vi "test 1.1.0 Mutation Adds Logging Section.vi"(8 "error in (no error)":errorcluster, 11 "TestCase in":refnum<class "Mutation.lvclass">) -> (0 "error out":errorcluster, 3 "TestCase out":refnum<class "Mutation.lvclass">)   [LabVIEW 2021, in "Mutation.lvclass"]
uses:
  Mutation.lvclass
  Mutation.lvclass/Mutation.ctl
  <vilib>/addons/_JKI Toolkits/VI Tester/TestCase.llb/TestCase.lvclass
  System Explorer/Implementation/Implementation.lvlib
  Scripting/Ballard/Ballard ARINC 429 Scripting.lvlib
  C:/Program Files/National Instruments/LabVIEW 2021/vi.lib/addons/_JKI Toolkits/VI Tester/TestCase.llb/TestCase.lvclass
  C:/Dev/CustomDevice/niveristand-ballard-arinc429-custom-device/Source/Custom Device Support/Tests/Unit/Mutation/Mutation.lvclass
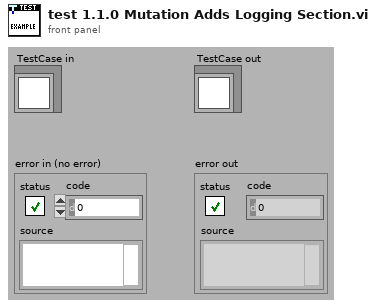
[diagram p1: front panel]
types:
  T1 = typedef "Custom Device API.lvlib/Custom Device Item Ref.ctl" = u64
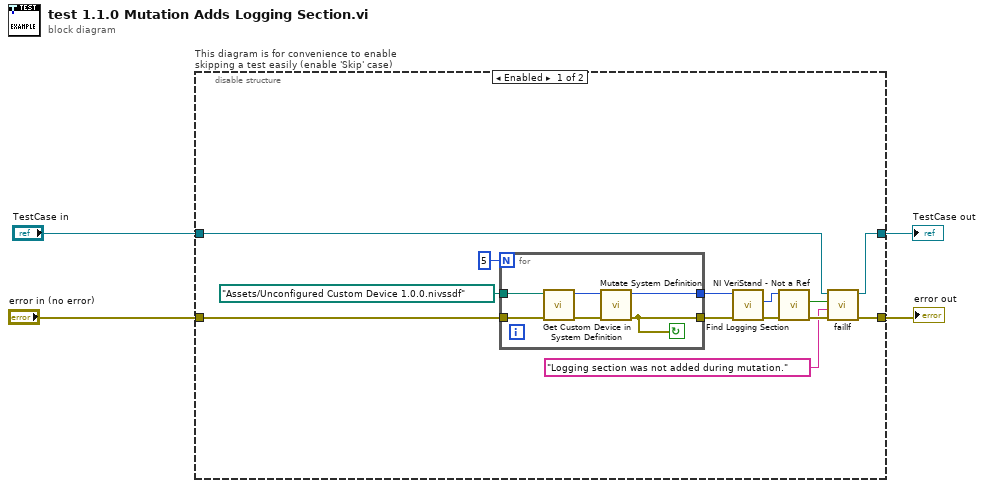
[diagram p0: block diagram]
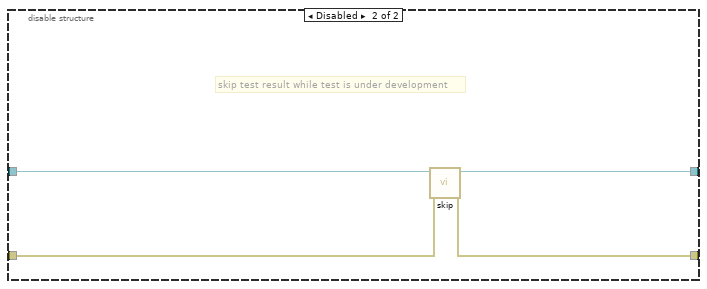
[diagram p2: hidden frame]
diagram:
  n1 = disable-structure "This diagram is for convenience to enable skipping a test easily (enable 'Skip' case)" shown="Enabled" {
    disable-tunnel: "TestCase in" -> [w9 w27]
    disable-tunnel: [w8 w25] -> w1
    disable-tunnel: [w10 w26] -> w3
    disable-tunnel: "error in (no error)" -> [w17 w24]
    frame Enabled {
      n2 = for {
        N: 5 -> [_]
        tunnel: path "Assets/Unconfigured Custom Device 1.0.0.nivssdf" ("Absolute or Relative Path") -> [w22]
        tunnel: [w19] -> w14
        tunnel: w17 -> [w23]
        tunnel: [w18] -> w15
        stop <- w18 continue-if-true
        n3 = call "Get Custom Device in System Definition.vi"("error in (no error)"=w23, "system definition"=w22) -> ("error out"=w21:errorcluster, "Ballard ARINC 429 custom device"=w20:u64)  [unwired: 8 in]
        n4 = call "Mutate System Definition.vi"("error in (no error)"=w21, "Device Ref in"=w20) -> ("error out"=w18:errorcluster, "Device Ref out"=w19:T1)  [unwired: 8 in]
      }
      n5 = call "Find Logging Section.vi"("error in"=w15, "Ballard ARINC 429 custom device in"=w14) -> ("error out"=w12:errorcluster, "logging"=w13:T1)  [unwired: 7 in, 1 out]
      n6 = call <vilib>:"NI VeriStand - Not a Ref.vi"("error in (no error)"=w12, "Item Ref"=w13) -> ("error out"=w11:errorcluster, "Not a Ref"=w7:bool)  [unwired: 7 in, 1 out]
      n7 = call-dynamic "failIf.vi"("error in (no error)"=w11, "message (\"\")"="Logging section was not added during mutation." ("message (\"\")"), "fail"=w7, "TestCase in"=w9) -> ("error out"=w10:errorcluster, "TestCase out"=w8:refnum<class "Mutation.lvclass">)  [unwired: 6 in]
    }
    frame Disabled {
      # "skip test result while test is under development"
      n8 = call <vilib>:"skip.vi"("error in (no error)"=w24, "TestCase in"=w27) -> ("error out"=w26:errorcluster, "TestCase out"=w25:refnum<class "Mutation.lvclass">)  [unwired: 8 in]
    }
  }
  "error out" <- w3
  "TestCase out" <- w1
